vi "CSM Target Timeout Error.vi"(8 "error in (no error)":errorcluster, 11 "Arguments (As CSM Name)":string) -> (0 "error out":errorcluster)   [LabVIEW 2017, in "Communicable State Machine.lvlib"]
doc: "Generates an error cluster describing a CSM \"Target Module Timeout\" error. A \"Target Module Timeout\" error occurs when the CSM attempts to send a synchronous message to a target module but does not receive a reply within the specified timeout period.\n\n-- <b>Controls</b> --\n- <b>Arguments (As CSM Name)</b>: Wired argument, passing the target module name."
uses:
  Communicable State Machine.lvlib
  AdvanceAPI/CSM - Keywords.vi
  _Shared/CSM Shared.lvlib
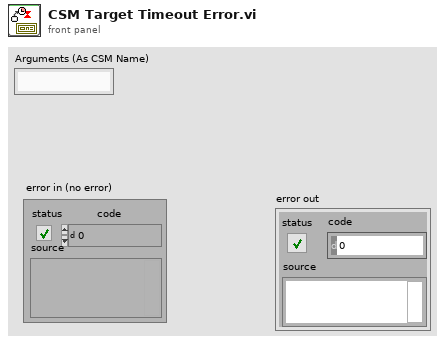
[diagram p1: front panel]
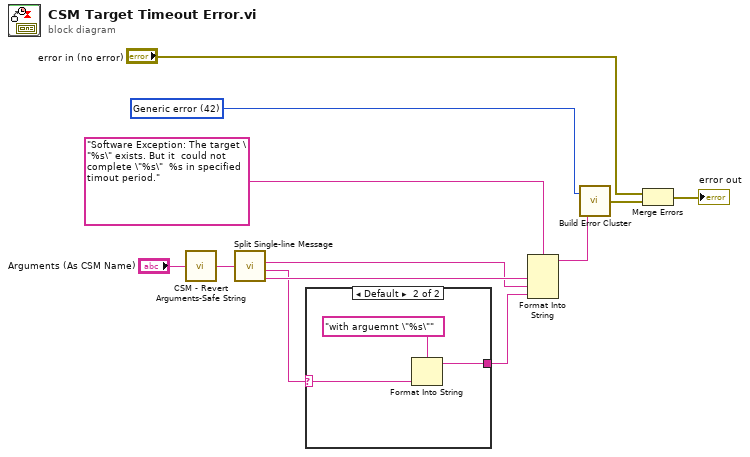
[diagram p0: block diagram]
diagram:
  w9 = 42 items=["No error", "Argument error", "Memory is full", "Out of zone", "End of file", "File already open", "Generic file I/O error", "File not found", "File permission error", "Disk is full", "Duplicate path", "Too many files open", "System feature not enabled", "Resource file not found", "Cannot add resource", "Resource not found", "Image not found", "Image memory error", "Pen does not exist", "Config type invalid", "Config token not found", "Config parse error", "Config memory error", "Bad external code format", "Bad external code offset", "External code not present", "Null window", "Destroy window error", "Null menu", "Print aborted", "Bad print record", "Print driver error", "Windows error during printing", "Memory error during printing", "Print dialog error", "Generic print error", "Invalid device refnum", "Device not found", "Device parameter error", "Device unit error", "Cannot open device", "Device call aborted", "Generic error", "Cancelled by user", "Object ID too low", "Object ID too high", "Object not in heap", "Unknown heap", "Unknown object (invalid DefProc)", "Unknown object (DefProc not in table)", "Message out of range", "Invalid (null) method", "Unknown message", "Manager call not supported", "Bad address", "Network operation in progress", "Network operation timed out", "Connection is busy", "Network attribute not supported", "Network error", "Address in use", "System out of memory", "Connection aborted", "Connection refused", "Not connected", "Already connected", "Connection closed", "Initialization error (interapplication manager)", "Bad occurrence", "Wait on unbound occurrence handler", "Occurrence queue overflow", "Datalog type conflict", "Unused", "Unrecognized type (interapplication manager)", "Memory corrupt", "Failed to make temporary DLL", "Old CIN version", "Drag socket not found", "Failed to load drop-object", "Failed to register OLE object", "Failed to release OLE object", "Format specifier type mismatch", "Unknown format specifier", "Too few format specifiers", "Too many format specifiers", "Scan failed", "Newer CIN version", "Error converting to variant", "Runtime menu error", "Password tampered", "Variant attribute not found", "Incompatible variant data type", "Event data is not available", "Event Store is not present", "Occurrence is not found", "Event Queue is not created", "Event info is not available", "Refnum passed is NULL", "Error retrieving Class GUID", "Error retrieving CoClass GUID", "Error retrieving TypeLib GUID.", "Bad built application magic bytes.", "Specific driver is different from the specific driver associated with the Logical Name.", "There is no session opened to the class driver.", "Max Error", "MAX - Error with config objects", "MAX - Error loading configuration", "MAX - Group not supported"]
  n1 = call "CSM - Revert Arguments-Safe String.vi"("Safe Argument String"="Arguments (As CSM Name)") -> ("Origin Argument String"=w5:string)  [unwired: 8 in]
  n2 = call "Split Single-line Message.vi"("single-line text"=w5) -> ("state"=w3:string, "args"=w2:string, "source/target"=w4:string)  [unwired: 6 in, 1 out]
  n3 = case shown="Default" w2 {
    selector: w2 -> [_ w15]
    tunnel: [_ w13] -> w1
    frame "" {
    }
    frame Default {
      n4 = Format Into String(format string="with arguemnt \"%s\"", w15) -> (resulting string=w13:string)  [unwired: 2 in, 1 out]
    }
  }
  n5 = Format Into String(format string="Software Exception: The target \"%s\" exists. But it  could not complete \"%s\"  %s in specified timout period." ("message"), w4, w3, w1) -> (resulting string=w10:string)  [unwired: 2 in, 1 out]
  n6 = call "Build Error Cluster.vi"("String to Prepend to Source (\"\")"=w10, "Code"=w9) -> ("error out"=w11:errorcluster)
  n7 = Merge Errors("error in (no error)", w11) -> (→"error out":errorcluster)
